vi "MoveObjectFast.vi"(8 "error in":errorcluster, 10 "Position":cluster{dbl, dbl}, 11 "GObj Refnum":refnum<vi>) -> (0 "error out":errorcluster, 3 "GObj Refnum dup":refnum<vi>)   [LabVIEW 2012]
doc: "Takes a GObject reference and moves the associated front panel terminal/decoration to the panel position specified. It does so in a loop with a small delay to provide a visual effect while remaining fast."
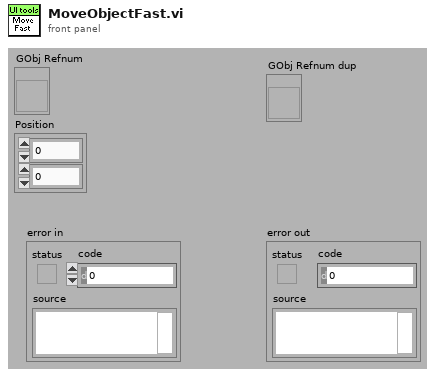
[diagram p1: front panel]
types:
  T1 = typedef "LVPositionTypeDef.ctl" = cluster{"Left":i32, "Top":i32}
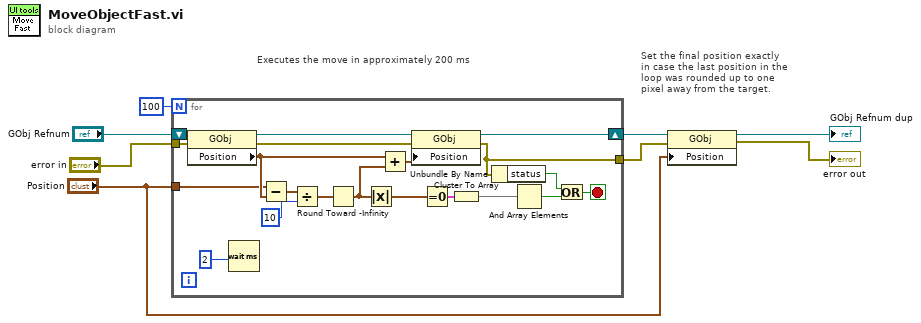
[diagram p0: block diagram]
diagram:
  # "Set the final position exactly\nin case the last position in the\nloop was rounded up to one\npixel away from the target."
  # "Executes the move in approximately 200 ms"
  n1 = for {
    N: 100 -> [_]
    tunnel: "Position" -> [w21]
    tunnel: "error in" -> [w20]
    shift-right: [w11] -> w5
    shift-left: "GObj Refnum" -> [w28]
    tunnel: [w10] -> w4
    stop <- w16 stop-if-true
    n2 = property class="GObj"(reference=w28, error in=w20) -> (reference out=w27:refnum<vi>, error out=w19:errorcluster, "Position"=w24:T1)
    n3 = Wait (ms)(milliseconds to wait=u32 2) -> ()  [unwired: 1 out]
    n4 = Subtract(x=w21, y=w24) -> (x-y=w23:cluster{dbl, dbl})
    n5 = Divide(x=w23, y=10) -> (x/y=w14:cluster{dbl, dbl})
    n6 = Round Toward -Infinity(1:w14) -> (0:w13:cluster{dbl, dbl})
    n7 = Absolute Value(x=w13) -> (abs(x)=w12:cluster{dbl, dbl})
    n8 = Add(x=w24, y=w13) -> (x+y=w15:cluster{dbl, dbl})
    n9 = property class="GObj"(reference=w27, error in=w19, "Position"=w15) -> (reference out=w11:refnum<vi>, error out=w10:errorcluster)
    n10 = Equal To 0?(x=w12) -> (x = 0?=w25:cluster{bool, bool})
    n11 = Cluster To Array(cluster=w25) -> (array=w26:bool[])
    n12 = Unbundle By Name(w10) -> ("status"=w17:bool)
    n13 = And Array Elements(Boolean array=w26) -> (logical AND=w18:bool)
    n14 = Or(x=w17, y=w18) -> (x .or. y?=w16:bool)
  }
  n15 = property class="GObj"(reference=w5, error in=w4, "Position"="Position") -> (reference out=→"GObj Refnum dup":refnum<vi>, error out=→"error out":errorcluster)
